vi "Adjust FIFO Size.vi"(8 "error in (no error)":errorcluster, 10 "New FIFO Instance Config":T1 {"Custom Data" format="%.0x"}, 11 "CIF_Iceoryx_PCAP_Universal in":refnum<class "CIF_Iceoryx_PCAP_Universal.lvclass">) -> (0 "error out":errorcluster, 3 "CIF_Iceoryx_PCAP_Universal out":refnum<class "CIF_Iceoryx_PCAP_Universal.lvclass">)   [LabVIEW 2021, in "CIF_Iceoryx_PCAP_Universal.lvclass"]
uses:
  CIF_Iceoryx_PCAP_Universal.lvclass
  D:/dev/Packages/CIF_Channels_Core/src/CIFChannels/CIFChannels.lvclass
  ChannelCommon/typedef/New FIFO Instance Configuration.ctl
  CIF_Iceoryx_PCAP_Universal.lvclass/CIF_Iceoryx_PCAP_Universal.ctl
  CIFChannels/CIFChannels.lvclass/CIFChannels.ctl
  ChannelCommon/typedef/Channel State.ctl
  ChannelCommon/typedef/Errors.ctl
  CIFChannels/Accessors/Read Channel State.vi
  ChannelCommon/Utilities/Add Error Core.vi
  ChannelCommon/ChannelCommon.lvlib
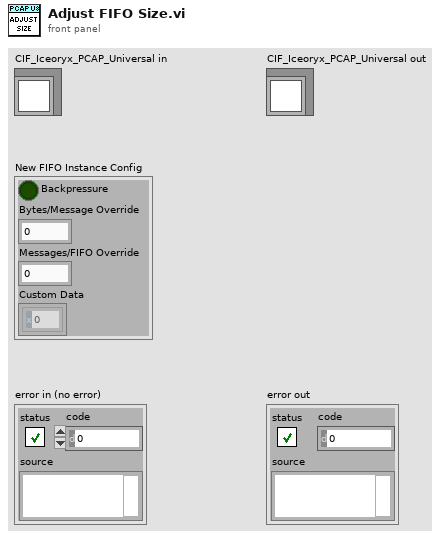
[diagram p1: front panel]
types:
  T1 = typedef "ChannelCommon.lvlib/New FIFO Instance Configuration.ctl" = cluster{"Backpressure":bool, "Bytes/Message Override":u32, "Messages/FIFO Override":u32, "Custom Data":u8[]}
  T2 = typedef "ChannelCommon.lvlib/Channel State.ctl" = enum8{"Creating", "Disconnected", "Connecting", "Connected", "Destroyed"}
  T3 = typedef "ChannelCommon.lvlib/Errors.ctl" = enum8{"gRPC Server Not Found", "Duplicate Channel", "Missing Channel", "Incorrect Type", "Flatten Error", "Unflatten Data", "Channel Length", "Plugin Connection", "gRPC Server Connection", "FIFO Unflatten", "Required Override", "Remove Not Found", "Multi Sub Not Supported", "Primary Already Connected", "Backpressure Not Supported", "Unable to Increase Buffer", "Data too Large"}
  T4 = typedef "CIF_Iceoryx_PCAP_Universal.lvclass/FIFO Configuration.ctl" = cluster{"Max Bytes":u32, "Best Effort Queue Depth":u32, "Best Effort Subscribers":u32, "Backpressure Queue Depth":u32, "Backpressure Subscribers":u32, "Linktype":u32}
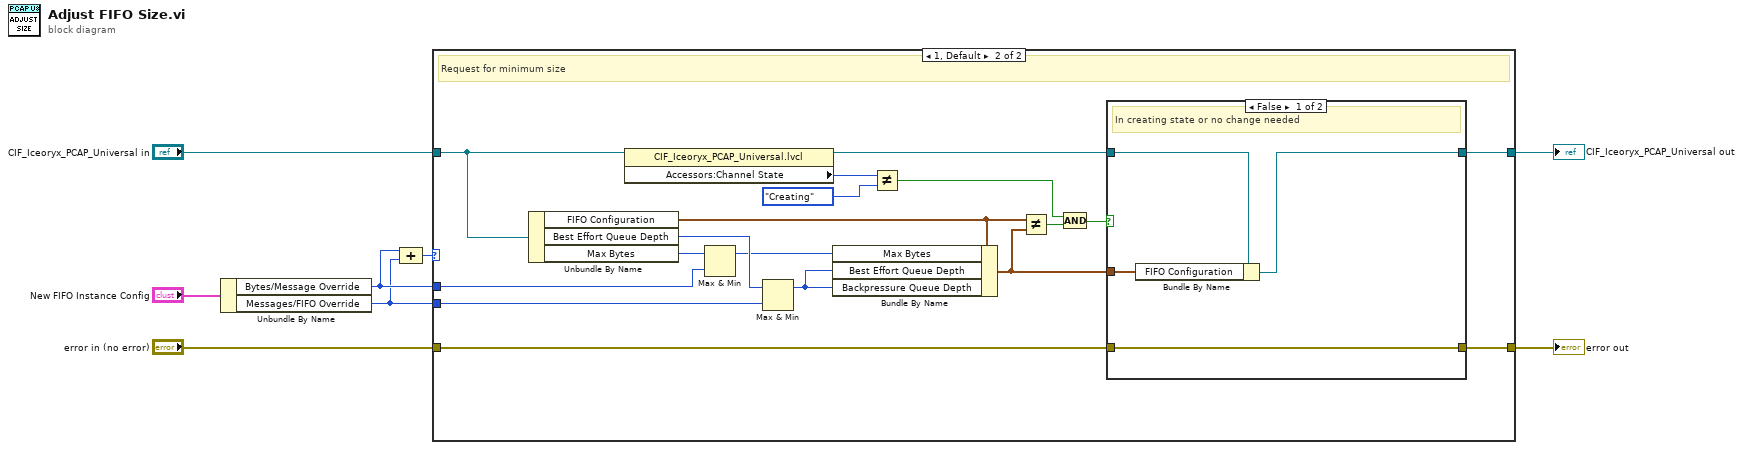
[diagram p0: block diagram]
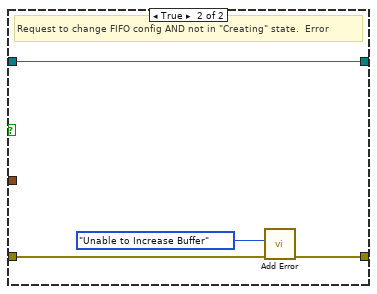
[diagram p3: hidden frame]
diagram:
  n1 = Unbundle By Name("New FIFO Instance Config") -> ("Bytes/Message Override"=w7:u32, "Messages/FIFO Override"=w6:u32)
  n2 = Compound Arithmetic op=ADD(w7, w6) -> (w8:u32)
  n3 = case shown="1, Default" w8 {
    tunnel: [w10 w11] -> w4
    tunnel: "CIF_Iceoryx_PCAP_Universal in" -> [w10 w22]
    tunnel: w7 -> [_ w28]
    tunnel: w6 -> [_ w27]
    tunnel: "error in (no error)" -> [w9 w17]
    tunnel: [w9 w16] -> w2
    frame 0 {
      # "No request for custom FIFO size"
    }
    frame 1, Default {
      # "Request for minimum size"
      n4 = Unbundle By Name(w22) -> ("FIFO Configuration"=w15:T4, "Best Effort Queue Depth"=w26:u32, "Max Bytes"=w25:u32)
      n5 = property class="CIF_Iceoryx_PCAP_Universal.lvcl"(reference=w22) -> (reference out=w12:refnum<class "CIF_Iceoryx_PCAP_Universal.lvclass">, "Accessors:Channel State"=w21:T2)  [unwired: 1 in, 1 out]
      n6 = Max & Min(x=w25, y=w28) -> (max(x,y)=w24:u32)  [unwired: 1 out]
      n7 = Max & Min(x=w26, y=w27) -> (max(x,y)=w23:u32)  [unwired: 1 out]
      n8 = Bundle By Name(cluster=w15, "Max Bytes"=w24, "Best Effort Queue Depth"=w23, "Backpressure Queue Depth"=w23) -> (w13:T4)
      n9 = Not Equal?(x=w21, y=Channel_State."Creating" ("Channel State")) -> (x != y?=w18:bool)
      n10 = Not Equal?(x=w15, y=w13) -> (x != y?=w19:bool)
      n11 = Compound Arithmetic op=AND(w18, w19) -> (w14:bool)
      n12 = case shown="False" w14 {
        tunnel: w17 -> [w29 w35]
        tunnel: [w29 w34] -> w16
        tunnel: w13 -> [w31 _]
        tunnel: w12 -> [w32 w33]
        tunnel: [w30 w33] -> w11
        frame False {
          # "In creating state or no change needed"
          n13 = Bundle By Name(cluster=w32, "FIFO Configuration"=w31) -> (w30:refnum<class "CIF_Iceoryx_PCAP_Universal.lvclass">)
        }
        frame True {
          # "Request to change FIFO config AND not in \"Creating\" state.  Error"
          n14 = call "Add Error.vi"("error in (no error)"=w35, "Error"=Errors."Unable to Increase Buffer") -> ("error out"=w34:errorcluster)  [unwired: 9 in]
        }
      }
    }
  }
  "CIF_Iceoryx_PCAP_Universal out" <- w4
  "error out" <- w2
